vi "Running Wrapper.vi"(8 "error in (no error)":errorcluster, 11 "CAN_Writer_NIXNET_Plugin in":refnum<class "CAN_Writer_CANsub_Plugin.lvclass">) -> (0 "error out":errorcluster, 2 "Destroy":bool, 3 "CAN_Writer_NIXNET_Plugin out":refnum<class "CAN_Writer_CANsub_Plugin.lvclass">)   [LabVIEW 2021, in "CAN_Writer_CANsub_Plugin.lvclass"]
uses:
  CAN_Writer_CANsub_Plugin.lvclass
  CAN_Writer_CANsub_Plugin.lvclass/CAN_Writer_CANsub_Plugin.ctl
  <vilib>/Platform/TimedLoop/XDataNode/wakeup.ctl
  <vilib>/Platform/TimedLoop/XDataNode/XDNodeRunTimeDep.lvlib
  <vilib>/Platform/TimedLoop/XDataNode/nitl_modes.ctl
  <vilib>/Platform/TimedLoop/XDataNode/timing_clust.ctl
  <vilib>/Platform/TimedLoop/XDataNode/XDataNode.xnode
  <vilib>/CIF Foundation/CIF Core/CIFCore/Class/CIFCorePlugin.lvclass
  C:/Program Files/National Instruments/LabVIEW 2021/vi.lib/CIF Foundation/CIF Core/CIFCore/Class/CIFCorePlugin.lvclass
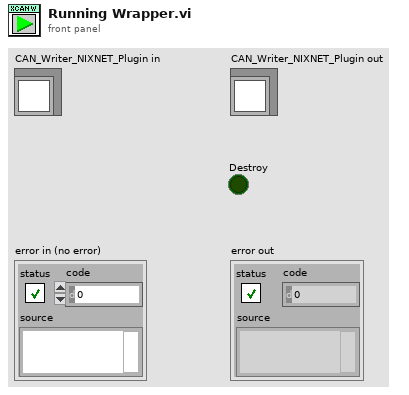
[diagram p1: front panel]
types:
  T1 = typedef "XDNodeRunTimeDep.lvlib/timing_clust.ctl" = cluster{"Expected End [f-1]":u64, "Actual End [f-1]":u64, "Finished Late? [f-1]":bool, "Expected End [i-1]":u64, "Actual End [i-1]":u64, "Finished Late? [i-1]":bool, "Expected Start [i]":u64, "Actual Start [i]":u64, "Expected Start [f]":u64, "Actual Start [f]":u64, "Source Name":string, "Structure Name":string, "Period":i64, "Deadline":i64, "Offset":i64, "Start":i64, "Priority":i32, "Timeout":i32, "Mode":T2, "Wakeup Reason":T3, "Error":errorcluster, "Source Type":string, "Secondary Source Type":string, "Global End Time":u64, "Global Start Time":u64, "Frame Duration":u64, "Iteration Duration":u64, "Assigned CPU":i32, "I/O Scan Engine Mode":u32}
  T2 = typedef "XDNodeRunTimeDep.lvlib/nitl_modes.ctl" = enum32{"No Change", "Process missed periods, maintain original phase", "Discard missed periods, maintain original phase", "Process missed periods, ignore original phase", "Discard missed periods, ignore original phase"}
  T3 = typedef "XDNodeRunTimeDep.lvlib/wakeup.ctl" = enum32{"Normal", "Aborted", "Asynchronous wakeup", "Timing source error", "Timed loop error", "Timeout"}
  T4 = typedef "CIFCorePlugin.lvclass/Running Internal Data.ctl" = cluster{"Refresh":bool, "Iterations":i64, "Housekeep only":bool, "Configured period (ns)":i64, "Update channel OOB":bool, "Configuration Change":bool, "Disable Auto Benchmark":bool, "gRPC Loop":bool, "Timed Loop Supported":bool, "Windows Late Cycle Warning":bool, "Prepared":bool}
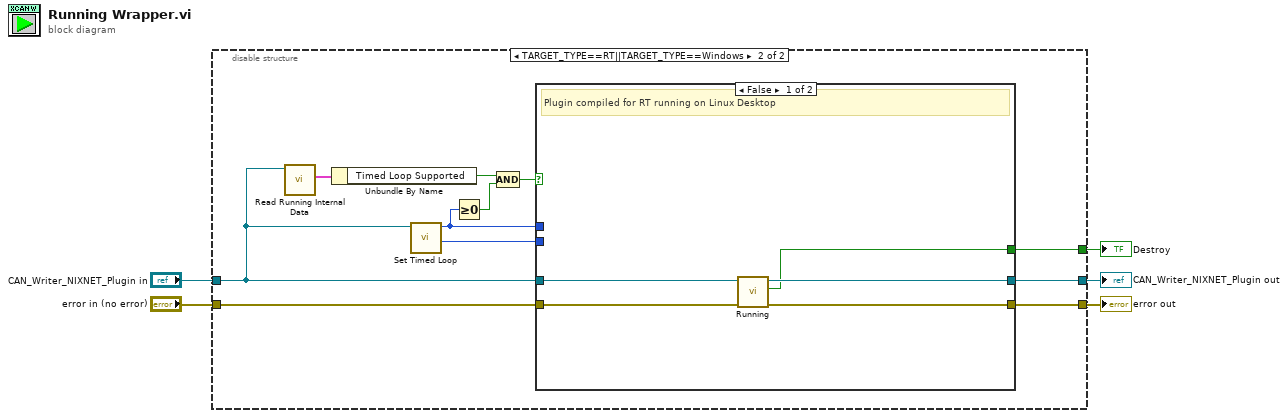
[diagram p0: block diagram]
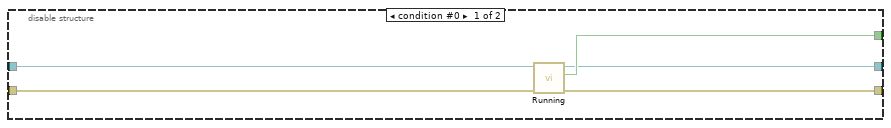
[diagram p2: hidden frame]
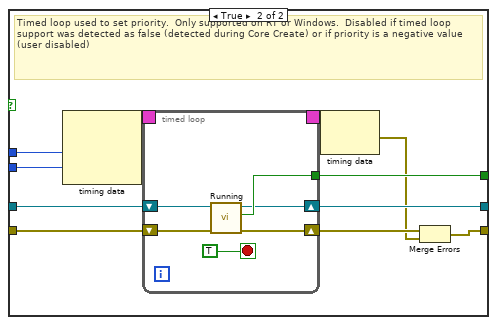
[diagram p3: hidden frame]
diagram:
  n1 = disable-structure shown="TARGET_TYPE==RT||TARGET_TYPE==Windows" {
    disable-tunnel: "CAN_Writer_NIXNET_Plugin in" -> [w6 w12]
    disable-tunnel: "error in (no error)" -> [w10 w21]
    disable-tunnel: [w8 w20] -> w5
    disable-tunnel: [w7 w19] -> w2
    disable-tunnel: [w9 w18] -> w1
    frame condition #0 {
      n2 = call "Running.vi"("error in (no error)"=w10, "CIFPlugin in"=w6) -> ("error out"=w9:errorcluster, "Destroy"=w8:bool, "CIFPlugin out"=w7:refnum<class "CAN_Writer_CANsub_Plugin.lvclass">)  [unwired: 7 in]
    }
    frame condition #1 (active) {
      n3 = call <vilib>:"Read Running Internal Data.vi"("CIFCorePlugin in"=w12) -> ("Running Internal Data"=w11:T4)  [unwired: 8 in, 2 out]
      n4 = Unbundle By Name(w11) -> ("Timed Loop Supported"=w15:bool)
      n5 = call <vilib>:"Set Timed Loop.vi"("CIFCorePlugin in"=w12) -> ("Processor"=w17:i32, "Priority"=w16:i32)  [unwired: 9 in]
      n6 = Greater Or Equal To 0?(x=w16) -> (x >= 0?=w14:bool)
      n7 = Compound Arithmetic op=AND(w15, w14) -> (w13:bool)
      n8 = case shown="False" w13 {
        tunnel: w21 -> [w25 w35]
        tunnel: [w22 w34] -> w20
        tunnel: [w24 w33] -> w19
        tunnel: [w23 w28] -> w18
        tunnel: w12 -> [w26 w32]
        tunnel: w16 -> [_ w31]
        tunnel: w17 -> [_ w30]
        frame False {
          # "Plugin compiled for RT running on Linux Desktop"
          n9 = call "Running.vi"("error in (no error)"=w25, "CIFPlugin in"=w26) -> ("error out"=w23:errorcluster, "Destroy"=w22:bool, "CIFPlugin out"=w24:refnum<class "CAN_Writer_CANsub_Plugin.lvclass">)  [unwired: 7 in]
        }
        frame True {
          # "Timed loop used to set priority.  Only supported on RT or Windows.  Disabled if timed loop support was detected as false (detected during Core Create) or if priority is a negative value (user disabled)"
          n10 = node-c288(w31, w30) -> (w37:T1)  [unwired: 1 in]
          n11 = timed-loop {
            timing: w37 -> [_]
            timing-out: [_] -> w36
            shift-right: [w38] -> w33
            shift-left: w32 -> [w42]
            shift-right: [w40] -> w29
            shift-left: w35 -> [w41]
            tunnel: [w39] -> w34
            stop <- TRUE stop-if-true
            n12 = call "Running.vi"("error in (no error)"=w41, "CIFPlugin in"=w42) -> ("error out"=w40:errorcluster, "Destroy"=w39:bool, "CIFPlugin out"=w38:refnum<class "CAN_Writer_CANsub_Plugin.lvclass">)  [unwired: 7 in]
          }
          n13 = node-c288(w36) -> (w27:errorcluster)
          n14 = Merge Errors(w29, w27) -> (w28:errorcluster)
        }
      }
    }
  }
  "error out" <- w1
  "CAN_Writer_NIXNET_Plugin out" <- w2
  "Destroy" <- w5
